vi "fake tool schema details.vi"(6 "mode":enum16{"slow", "fast"}(ring)=enum."fast", 7 "count":i32=3, 8 "config":T1, 9 "voltage":dbl[unit], 10 "setpoint":dbl=25.0 min=0.0 max=100.0, 11 "level":u8=7) -> (0 "config out":T1, 1 "voltage out":dbl[unit], 2 "setpoint out":dbl, 3 "level out":u8, 4 "mode out":enum16{"slow", "fast"}(ring), 5 "count out":i32)   [LabVIEW 2020, in "MCP Server tests.lvlib"]
doc: "Fake tool to test the details tools/list gives about each input beyond its type: the descriptions of cluster elements at any depth (also inside an array of clusters), the value range of integers from their representation, the data entry limits of numeric controls, the unit of a numeric with a unit, and the default value of inputs that are not required. Each input is returned unchanged on an output."
uses:
  MCP Server tests.lvlib
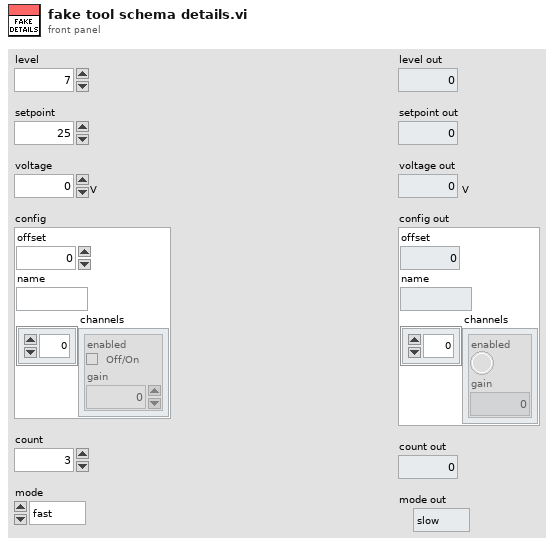
[diagram p1: front panel]
types:
  T1 = cluster{"offset":i16, "name":string, "channels":cluster{"enabled":bool, "gain":dbl}[]}
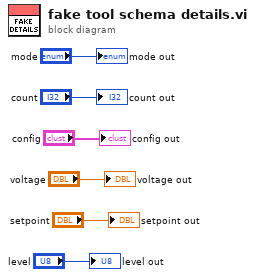
[diagram p0: block diagram]
diagram:
  "level out" <- "level"
  "setpoint out" <- "setpoint"
  "voltage out" <- "voltage"
  "config out" <- "config"
  "count out" <- "count"
  "mode out" <- "mode"
